vi "Generate New Overlay.vi"(4 "Pixellate":bool, 6 "Label?":bool, 8 "error in":errorcluster, 10 "Lithography Data":T2(array[cluster]), 11 "BigMAQ in":refnum<class "BigMAQ.lvclass">) -> (0 "error out":errorcluster, 3 "BigMAQ out":refnum<class "BigMAQ.lvclass">)   [LabVIEW 2019, in "BigMAQ.lvclass"]
uses:
  BigMAQ.lvclass
  <userlib>/LevyLab/Relay Box/Typedefs/Resistor--enum.ctl
  BigMAQ.lvclass/BigMAQ.ctl
  <userlib>/LevyLab/Relay Box/Relay-Box.lvclass
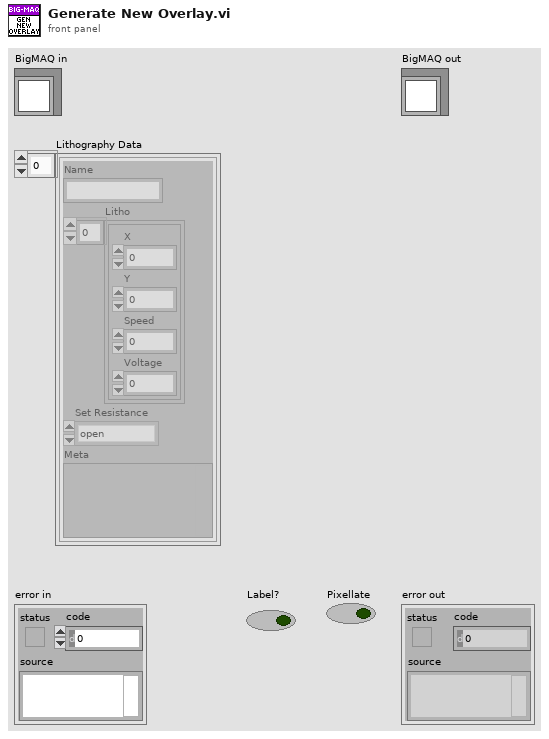
[diagram p1: front panel]
types:
  T1 = typedef "Relay-Box.lvclass/Resistor--enum.ctl" = enum16{"open", "discharge tip", "0 ohms", "100k ohm", "10M ohm", "1G ohm"}
  T2 = cluster{"Name":string, "Litho":cluster{"X":dbl, "Y":dbl, "Speed":dbl, "Voltage":dbl}[], "Set Resistance":T1, "Meta":variant}[]
  T3 = typedef "IMAQ Image.ctl" = refnum<image>
  T4 = typedef "BigMAQ.lvclass/Overlay.ctl" = cluster{"Name":string, "Data":cluster{"Points":cluster{"X":dbl, "Y":dbl}[], "Voltages":dbl[]}, "Changes":cluster{"MD5 Digest":string, "Changed?":bool}}
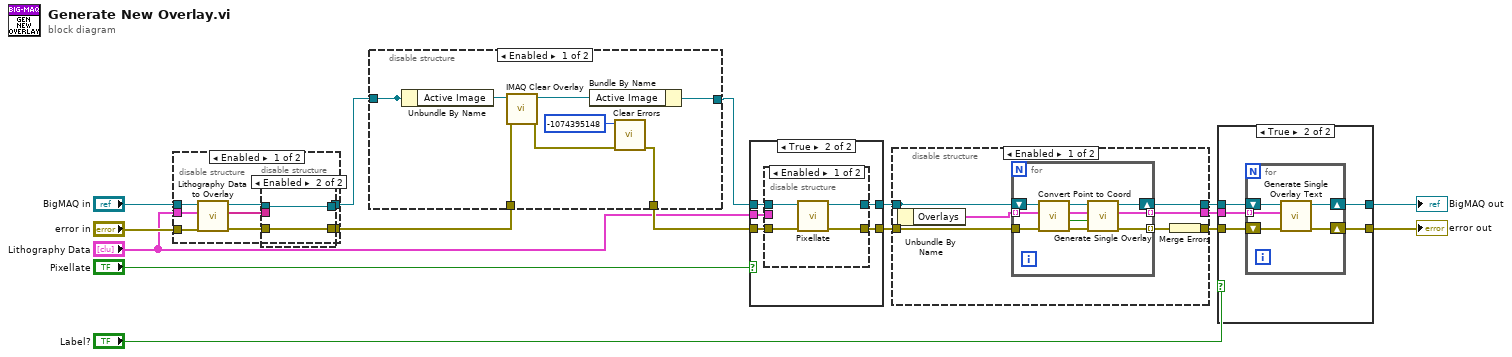
[diagram p0: block diagram]
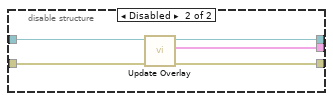
[diagram p3: hidden frame]
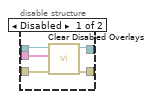
[diagram p4: hidden frame]
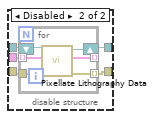
[diagram p7: hidden frame]
diagram:
  n1 = disable-structure shown="Enabled" {
    disable-tunnel: "BigMAQ in" -> [w24 w33]
    disable-tunnel: "error in" -> [w23 w32]
    disable-tunnel: [w19 w32] -> w7
    disable-tunnel: [w18 w33] -> w2
    disable-tunnel: "Lithography Data" -> [w17 _]
    frame Enabled {
      n2 = call "Lithography Data to Overlay.vi"("error in"=w23, "Lithography Data"=w17, "BigMAQ in"=w24) -> ("error out"=w21:errorcluster, "Disabled Overlays"=w20:string[], "BigMAQ out"=w22:refnum<class "BigMAQ.lvclass">)  [unwired: 6 in]
      n3 = disable-structure shown="Enabled" {
        disable-tunnel: w22 -> [w29 w31]
        disable-tunnel: w21 -> [w28 w30]
        disable-tunnel: w20 -> [w27 _]
        disable-tunnel: [w26 w30] -> w19
        disable-tunnel: [w25 w31] -> w18
        frame Disabled {
          n4 = call "Clear Disabled Overlays.vi"("error in"=w28, "Disabled Overlays"=w27, "BigMAQ in"=w29) -> ("error out"=w26:errorcluster, "BigMAQ out"=w25:refnum<class "BigMAQ.lvclass">)  [unwired: 7 in]
        }
        frame Enabled {
        }
      }
    }
    frame Disabled {
    }
  }
  n5 = disable-structure shown="Enabled" {
    disable-tunnel: [w34 w43] -> w1
    disable-tunnel: w7 -> [w39 w42]
    disable-tunnel: w2 -> [w38 w43]
    disable-tunnel: [w35 w42] -> w6
    frame Enabled {
      n6 = Unbundle By Name(w38) -> ("Active Image"=w41:T3)
      n7 = call "IMAQ Clear Overlay"("error in (no error)"=w39, "Image"=w41) -> ("error out"=w36:errorcluster, "Image Out"=w40:T3)  [unwired: 8 in]
      n8 = Bundle By Name(cluster=w38, "Active Image"=w40) -> (w34:refnum<class "BigMAQ.lvclass">)
      n9 = call <vilib>:"Clear Errors.vi"("error in (no error)"=w36, "specific error code to clear (0: all)"=-1074395148) -> ("error out"=w35:errorcluster)  [unwired: 4 in, 1 out]
    }
    frame Disabled {
    }
  }
  n10 = case shown="True" "Pixellate" {
    tunnel: [w44 w50] -> w8
    tunnel: [w45 w49] -> w3
    tunnel: w1 -> [w45 w48]
    tunnel: w6 -> [w44 w47]
    tunnel: "Lithography Data" -> [_ w46]
    frame False {
    }
    frame True {
      n11 = disable-structure shown="Enabled" {
        disable-tunnel: [w54 w56] -> w50
        disable-tunnel: [w53 w58] -> w49
        disable-tunnel: w48 -> [w52 w59]
        disable-tunnel: w47 -> [w51 w57]
        disable-tunnel: w46 -> [_ w55]
        frame Enabled {
          n12 = call "Pixellate.vi"("error in"=w51, "BigMAQ in"=w52) -> ("error out"=w54:errorcluster, "BigMAQ out"=w53:refnum<class "BigMAQ.lvclass">)  [unwired: 8 in]
        }
        frame Disabled {
          n13 = for {
            shift-right: [w64] -> w58
            shift-left: w59 -> [w65]
            tunnel: w57 -> [w63]
            tunnel: [w62] -> w56 mode=indexing
            tunnel: [w61] -> _ mode=indexing
            tunnel: w55 -> [w60] mode=indexing
            n14 = call "Pixellate Lithography Data.vi"("error in"=w63, "Lithography Data"=w60, "BigMAQ in"=w65) -> ("error out"=w62:errorcluster, "Array"=w61:T4[], "BigMAQ out"=w64:refnum<class "BigMAQ.lvclass">)  [unwired: 6 in]
          }
        }
      }
    }
  }
  n15 = disable-structure shown="Enabled" {
    disable-tunnel: [w71 w86] -> w14
    disable-tunnel: [w70 w84] -> w12
    disable-tunnel: [w69 w85] -> w9
    disable-tunnel: w8 -> [w68 w83]
    disable-tunnel: w3 -> [w67 w87]
    frame Enabled {
      n16 = Unbundle By Name(w67) -> ("Overlays"=w66:T4[])
      n17 = for {
        tunnel: w66 -> [w76] mode=indexing
        tunnel: w68 -> [w74]
        tunnel: [w81] -> w72 mode=indexing
        shift-right: [w82] -> w71
        shift-left: w67 -> [w79]
        tunnel: [w80] -> w69 mode=indexing
        n18 = call "Convert Point to Coord.vi"("error in"=w74, "Overlay"=w76, "BigMAQ in"=w79) -> ("error out"=w75:errorcluster, "Voltage Constant?"=w73:bool, "output cluster"=w77:T4, "BigMAQ out"=w78:refnum<class "BigMAQ.lvclass">)  [unwired: 5 in]
        n19 = call "Generate Single Overlay.vi"("error in"=w75, "Single Color"=w73, "Overlay"=w77, "BigMAQ in"=w78) -> ("error out"=w81:errorcluster, "Overlay Out"=w80:T4, "BigMAQ out"=w82:refnum<class "BigMAQ.lvclass">)  [unwired: 4 in, 1 out]
      }
      n20 = Merge Errors(w72) -> (w70:errorcluster)
    }
    frame Disabled {
      n21 = call "Update Overlay.vi"("error in"=w83, "BigMAQ in"=w87) -> ("error out"=w84:errorcluster, "Overlays"=w85:T4[], "BigMAQ out"=w86:refnum<class "BigMAQ.lvclass">)  [unwired: 7 in]
    }
  }
  n22 = case shown="True" "Label?" {
    tunnel: w14 -> [w89 w94]
    tunnel: [w89 w93] -> w13
    tunnel: w12 -> [w88 w92]
    tunnel: [w88 w91] -> w11
    tunnel: w9 -> [_ w90]
    frame False {
    }
    frame True {
      n23 = for {
        tunnel: w90 -> [w95] mode=indexing
        shift-right: [w98] -> w93
        shift-left: w94 -> [w99]
        shift-right: [w96] -> w91
        shift-left: w92 -> [w97]
        n24 = call "Generate Single Overlay Text.vi"("error in"=w97, "Overlay"=w95, "BigMAQ in"=w99) -> ("error out"=w96:errorcluster, "BigMAQ out"=w98:refnum<class "BigMAQ.lvclass">)  [unwired: 7 in]
      }
    }
  }
  "error out" <- w11
  "BigMAQ out" <- w13
